vi "CIF Publisher from Refnum.vi"(3 "CIF Publisher Refnum":T1 {"refnum" format="%.0x"}) -> (5 "CIF Publisher U64":u64)   [LabVIEW 2021, in "Iceoryx.lvlib"]
uses:
  Typedef/CIF Publisher Refnum.ctl
  Iceoryx.lvlib
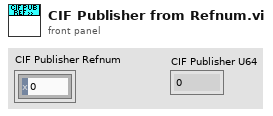
[diagram p1: front panel]
types:
  T1 = typedef "Iceoryx.lvlib/CIF Publisher Refnum.ctl" = cluster{"refnum":u64}
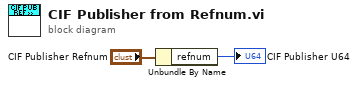
[diagram p0: block diagram]
diagram:
  n1 = Unbundle By Name("CIF Publisher Refnum") -> ("refnum"=→"CIF Publisher U64":u64)
